vi "AutoHelper_DelayedAction.vi"(6 "Pass_Through_Time":dbl=-1.0 format="%33.4f", 9 "Delay Time Sec":dbl, 11 "New Step":bool) -> (0 "Timeout ALT":bool, 1 "Remaining Delay Time Sec":dbl, 2 "Delayed Action Pulse":bool, 3 "Delayed Action":bool, 4 "Remaining ALT":dbl)   [LabVIEW 2019, in "Trajectory_Library.lvlib"]
doc: "Implements a simplified state machine similar to a mechanical / electrical drum sequencer. When the Drum Sequencer is \"Ready\" and the \"Initiate\" input becomes TRUE,, the drum sequences through its set of steps from 1 to N. After each Step is executed it is followed by a wait. During the wait the Step output indicates \"Do Nothing\". The number of Steps is determined by the number of elements in the \"Step Times\" input array. Once all the steps have been executed, the Drum Sequencer cycles bac to wait for another initiate. \n\nThere is a Cancel input that interrupts the sequence, executes the Cancel Step, performs the cancel wait, and then returns to wait for an Initiate action. \n\nIf any of the Step Times, or Cancel times are negative, or there more than 32 steps, or less than 1 step an error is signaled. The drum sequencer selects the error state and stays there.\n\nInputs:\n\nOutputs:"
uses:
  Trajectory_Library.lvlib
  Util_GetTime_U32.vi
  Util_GetTime_U64.vi
  <vilib>/Utility/semaphor.llb/Obtain Semaphore Reference.vi
  Timer_Reset.vi
  Timer_Start.vi
  Timer_Stop.vi
panel:
  # "For Debug"
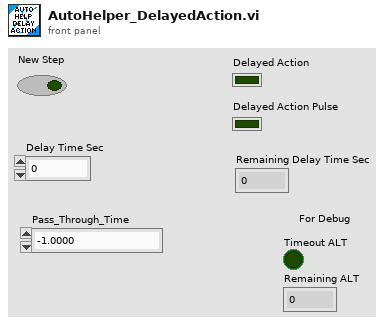
[diagram p1: front panel]
types:
  T1 = typedef "Trajectory_Library.lvlib/TIMER.ctl" = cluster{"StartTime":dbl, "Accumulated TIme":dbl, "Running":bool, "semaphore":T2}
  T2 = typedef "Semaphore RefNum" = refnum<k1>
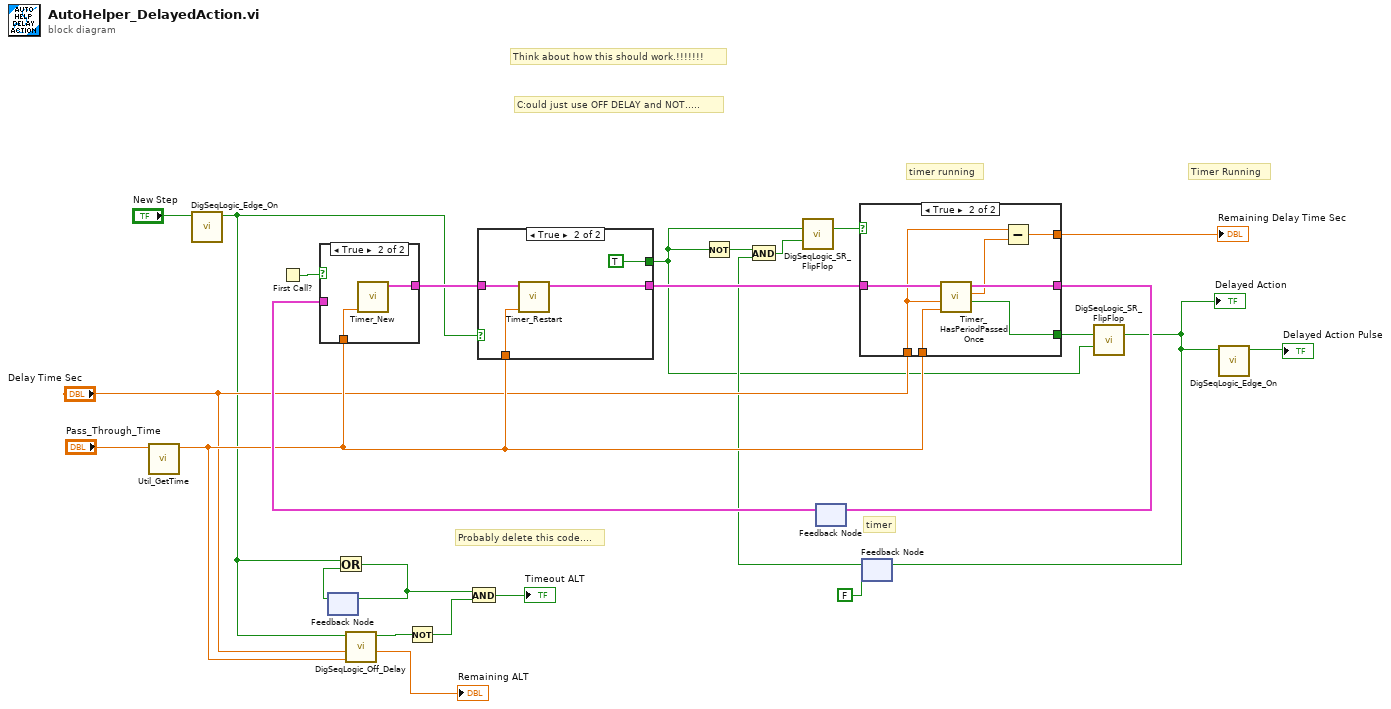
[diagram p0: block diagram]
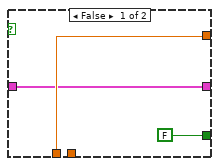
[diagram p2: hidden frame]
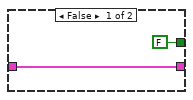
[diagram p3: hidden frame]
diagram:
  # "Probably delete this code...."
  # "Think about how this should work.!!!!!!!"
  # "C:ould just use OFF DELAY and NOT....."
  # "timer running"
  # "Timer Running"
  # "timer"
  n1 = call "Util_GetTime.vi"("Pass_Through_Time"="Pass_Through_Time") -> ("FPGA_Time_Seconds"=w16:dbl)  [unwired: 8 in, 2 out]
  n2 = call "DigSeqLogic_Edge_On.vi"("Input"="New Step") -> ("On Edge"=w11:bool)  [unwired: 10 in]
  n3 = First Call?() -> (First Call?: T/F=w24:bool)
  n4 = feedback #1() -> (w12:bool)  [unwired: 1 in]
  n5 = Or(x=w11, y=w12) -> (x .or. y?=w8:bool)
  n6 = feedback-in #1(w8) -> ()
  n7 = call "DigSeqLogic_Off_Delay.vi"("Time"=w16, "Delay"="Delay Time Sec", "Input"=w11) -> ("Remain"=→"Remaining ALT":dbl, "Output"=w14:bool)  [unwired: 7 in]
  n8 = Not(x=w14) -> (.not. x?=w10:bool)
  n9 = And(x=w8, y=w10) -> (x .and. y?=→"Timeout ALT":bool)
  n10 = feedback #2() -> (w23:T1)  [unwired: 1 in]
  n11 = case shown="True" w24 {
    tunnel: [w27 w29] -> w22
    tunnel: w16 -> [_ w28]
    tunnel: w23 -> [w27 _]
    frame False {
    }
    frame True {
      n12 = call "Timer_New.vi"("Pass_Through_Time"=w28) -> ("TIMER"=w29:T1)  [unwired: 10 in]
    }
  }
  n13 = case shown="True" w11 {
    tunnel: [w31 w35] -> w21
    tunnel: w22 -> [w31 w34]
    tunnel: w16 -> [_ w33]
    tunnel: [FALSE TRUE] -> w2
    frame False {
    }
    frame True {
      n14 = call "Timer_Restart.vi"("Pass_Through_Time"=w33, "in Timer"=w34) -> ("out Timer"=w35:T1)  [unwired: 9 in]
    }
  }
  n15 = Not(x=w2) -> (.not. x?=w4:bool)
  n16 = feedback #3(FALSE ("Expired")) -> (w3:bool)
  n17 = And(x=w4, y=w3) -> (x .and. y?=w1:bool)
  n18 = call "DigSeqLogic_SR_FlipFlop.vi"("Set"=w2, "Reset"=w1) -> ("Output"=w18:bool)  [unwired: 12 in, 1 out]
  n19 = case shown="True" w18 {
    tunnel: w21 -> [w37 w45]
    tunnel: w16 -> [_ w44]
    tunnel: [w37 w43] -> w20
    tunnel: "Delay Time Sec" -> [w38 w42]
    tunnel: [w38 w40] -> w19
    tunnel: [FALSE ("Expired") w39] -> w7
    frame False {
    }
    frame True {
      n20 = call "Timer_HasPeriodPassedOnce.vi"("Pass_Through_Time"=w44, "Period"=w42, "in Timer"=w45) -> ("Expired"=w39:bool, "CurrentTImer"=w41:dbl, "out Timer"=w43:T1)  [unwired: 6 in]
      n21 = Subtract(x=w42, y=w41) -> (x-y=w40:dbl)
    }
  }
  "Remaining Delay Time Sec" <- w19
  n22 = feedback-in #2(w20) -> ()
  n23 = call "DigSeqLogic_SR_FlipFlop.vi"("Set"=w7, "Reset"=w2) -> ("Output"=w6:bool)  [unwired: 12 in, 1 out]
  "Delayed Action" <- w6
  n24 = feedback-in #3(w6) -> ()
  n25 = call "DigSeqLogic_Edge_On.vi"("Input"=w6) -> ("On Edge"=→"Delayed Action Pulse":bool)  [unwired: 10 in]
